vi "Migrate Dependencies.vi"(0 "Project path":path=path "C:/Workspace/measurement-migration-tool/src/Test Folder/Shared Test/Shared Test.lvproj", 5 "Measurement paths":path[](array[path]), 7 "Plug-in names":string[](array[string]), 9 "Progress":refnum<vi>, 11 "error in":errorcluster) -> (4 "Instrument containing subVIs":path[][](array[path]), 15 "error out":errorcluster)   [LabVIEW 2021, in "Multiple Migrator.lvlib"]
doc: "Migrate multiple measurements along with their dependencies, either dependencies being shared among measurements or measurements having their own depenencies."
uses:
  Multiple Migrator.lvlib
panel:
  # "Dependencies Migration"
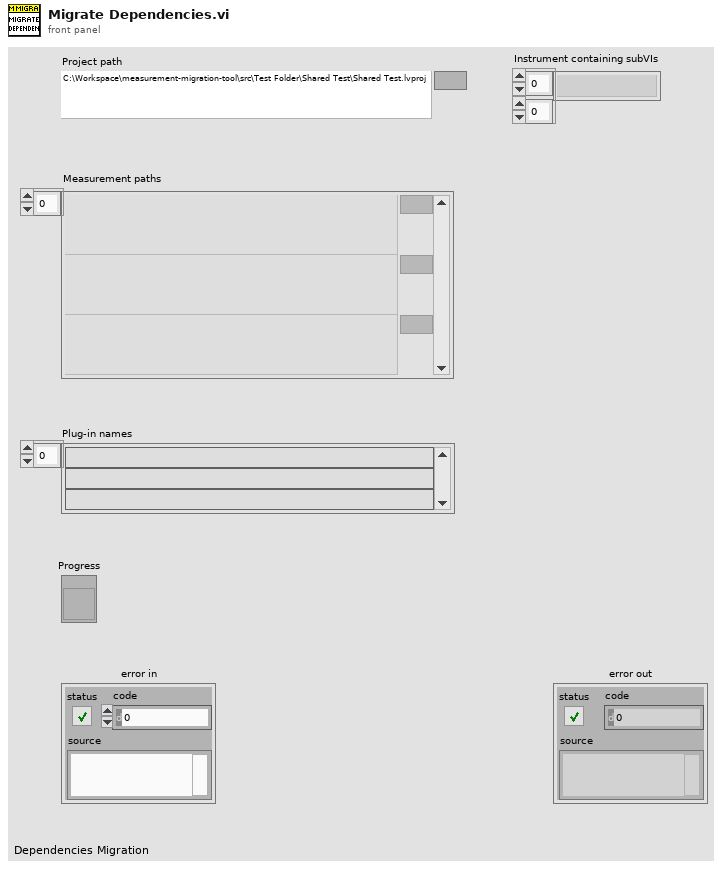
[diagram p1: front panel]
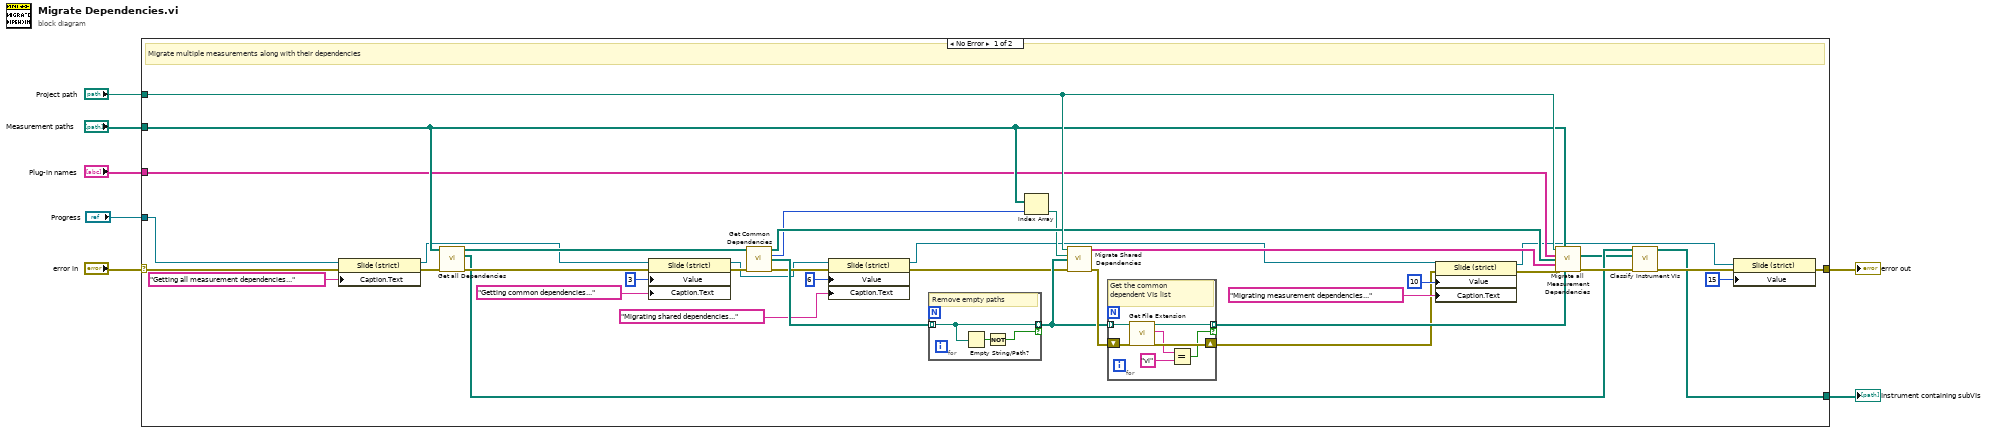
[diagram p0: block diagram]
diagram:
  n1 = case shown="No Error" "error in" {
    selector: "error in" -> [w34 w57]
    tunnel: "Project path" -> [w46 _]
    tunnel: "Measurement paths" -> [w45 _]
    tunnel: "Plug-in names" -> [w44 _]
    tunnel: [w15 w57] -> w4
    tunnel: [w9 _] -> w2
    tunnel: "Progress" -> [w32 _]
    frame No Error {
      # "Migrate multiple measurements along with their dependencies"
      n2 = property class="Slide (strict)"(reference=w32, error in=w34, "Caption.Text"="Getting all measurement dependencies...") -> (reference out=w27:refnum<vi>, error out=w33:errorcluster)
      n3 = call "Get all Dependencies.vi"("Measurement paths"=w45, "error in (no error)"=w33) -> ("All dependencies"=w43:path[][], "Instrument containing subVIs"=w10:path[][], "error out"=w30:errorcluster)  [unwired: 11 in]
      n4 = property class="Slide (strict)"(reference=w27, error in=w30, "Value"=3, "Caption.Text"="Getting common dependencies...") -> (reference out=w21:refnum<vi>, error out=w29:errorcluster)
      n5 = call "Get Common Dependencies.vi"("All dependencies"=w43, "error in (no error)"=w29) -> ("Measurement dependencies"=w42:path[][], "Measurement index"=w36:i32, "Common dependencies"=w37:path[], "error out"=w23:errorcluster)  [unwired: 10 in]
      n6 = property class="Slide (strict)"(reference=w21, error in=w23, "Value"=6, "Caption.Text"="Migrating shared dependencies...") -> (reference out=w14:refnum<vi>, error out=w22:errorcluster)
      n7 = for {
        tunnel: [w47] -> w35 mode=indexing if=w48
        tunnel: w37 -> [w47] mode=indexing
        # "Remove empty paths"
        n8 = Empty String/Path?(string/path=w47) -> (empty?=w49:bool)
        n9 = Not(x=w49) -> (.not. x?=w48:bool)
      }
      n10 = Index Array(array=w45, index=w36) -> (element=w38:path)
      n11 = call "Migrate Shared Dependencies.vi"("Project path"=w46, "Measurement path"=w38, "Common dependencies"=w35, "error in (no error)"=w22) -> ("Outside items"=w41:string[], "error out"=w39:errorcluster)  [unwired: 10 in]
      n12 = for {
        shift-right: [w55] -> w18
        shift-left: w39 -> [w56]
        tunnel: [w51] -> w40 mode=indexing if=w52
        tunnel: w35 -> [w50] mode=indexing
        # "Get the common dependent VIs list"
        n13 = call <vilib>:"Get File Extension.vi"("error in (no error)"=w56, "file"=w50) -> ("error out"=w55:errorcluster, "lowercase file extension"=w53:string, "dup file"=w51:path)  [unwired: 5 in, 2 out]
        n14 = Equal?(x=w53, y="vi" ("x")) -> (x = y?=w52:bool)
      }
      n15 = property class="Slide (strict)"(reference=w14, error in=w18, "Value"=10, "Caption.Text"="Migrating measurement dependencies...") -> (reference out=w13:refnum<vi>, error out=w17:errorcluster)
      n16 = call "Migrate all Measurement Dependencies.vi"("Project path"=w46, "Measurement paths"=w45, "Plug-in names"=w44, "Measurement dependencies"=w42, "Outside items"=w41, "error in (no error)"=w17, "Shared dependent VIs"=w40) -> ("DestinationDirectory"=w8:path[], "error out"=w12:errorcluster)  [unwired: 7 in]
      n17 = call "Classify Instrument VIs.vi"("InstrContaining"=w10, "DestinationDirectory"=w8, "error in (no error)"=w12) -> ("InstrContainingVI[]"=w9:path[][], "error out"=w11:errorcluster)  [unwired: 11 in]
      n18 = property class="Slide (strict)"(reference=w13, error in=w11, "Value"=15) -> (error out=w15:errorcluster)  [unwired: 1 out]
    }
    frame Error {
    }
  }
  "error out" <- w4
  "Instrument containing subVIs" <- w2
